vi "Own20261012_PublicSetNodeLabel_v1.vi"() -> ()   [LabVIEW 2024]
panel:
  out "error out":errorcluster caption="错误输出"
  in  "label":string
  in  "node_id":u32
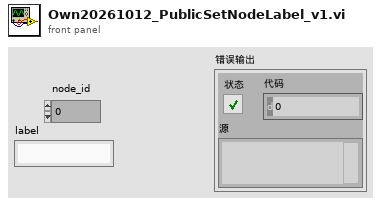
[diagram p1: front panel]
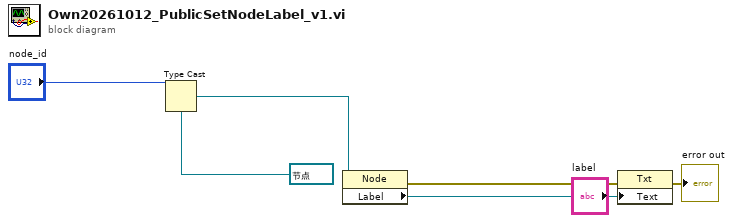
[diagram p0: block diagram]
diagram:
  n1 = Type Cast(type=refnum<vi> refnum ("引用"), x="node_id") -> (*(type *) &x=w5:refnum<vi>)
  n2 = property class="Node"(reference=w5) -> (error out=w3:errorcluster, "Label"=w4:refnum<vi>)  [unwired: 1 in, 1 out]
  n3 = property class="Txt"(reference=w4, error in=w3, "Text"="label") -> (error out=→"error out":errorcluster)  [unwired: 1 out]
